vi "Progress Bar Example with User Cancel.vi"() -> ()   [LabVIEW 2015]
doc: "This example VI illustrates how to implement the process to handle situation when user cancels the operations."
uses:
  Library/New Job Status.vi
  Library/New Item Status.vi
  Library/Class/Finish.vi
  Library/Simple Progress Bar.lvlib
  Library/Class/Bar.lvclass
panel:
  out "Process Error":errorcluster
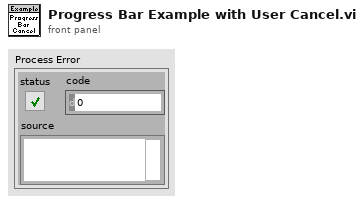
[diagram p1: front panel]
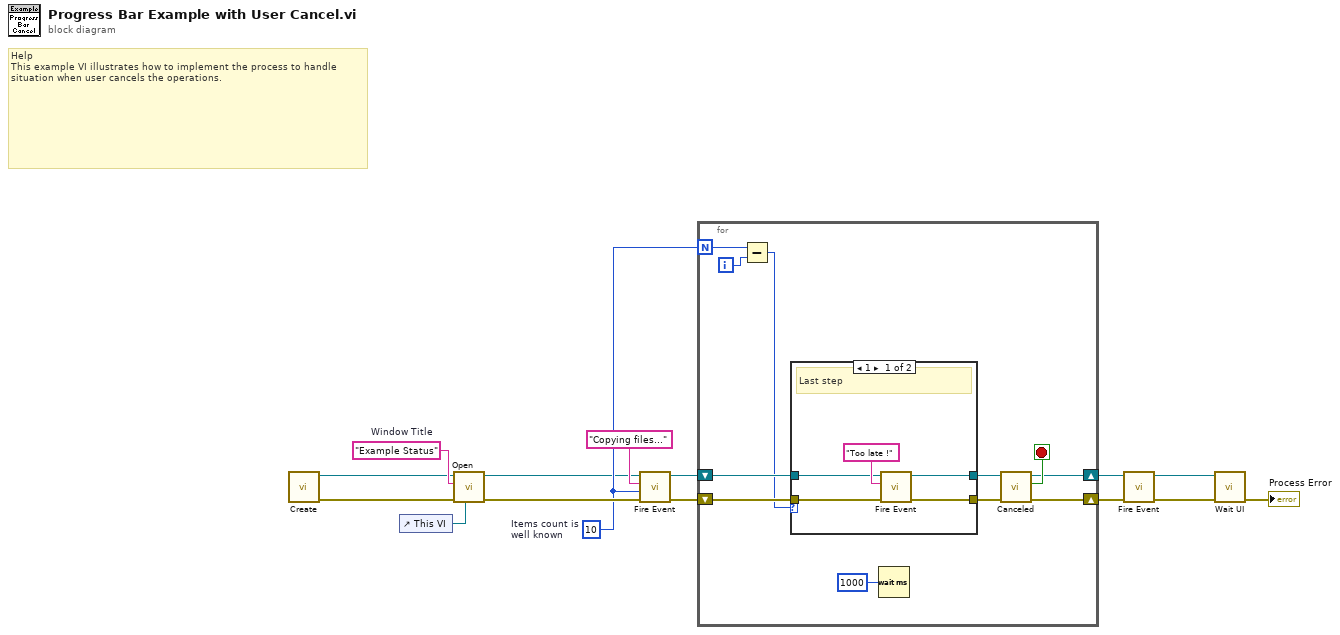
[diagram p0: block diagram]
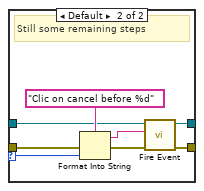
[diagram p2: hidden frame]
diagram:
  w10 = 10  # Items count is  well known
  w14 = "Example Status"  # Window Title
  # "Help\nThis example VI illustrates how to implement the process to handle situation when user cancels the operations."
  n1 = call "Create.vi"() -> ("error out"=w15:errorcluster, "Bar out"=w3:refnum<class "Bar.lvclass">)  [unwired: 10 in]
  n2 = control-ref of="This VI"() -> (w4:refnum<vi>)
  n3 = call "Open.vi"("Caller VI"=w4, "error in (no error)"=w15, "Window Title"=w14, "Bar in"=w3) -> ("error out"=w13:errorcluster, "Bar out"=w2:refnum<class "Bar.lvclass">)  [unwired: 6 in]
  n4 = call-poly "Fire Event.vi"("error in (no error)"=w13, "Items Count (unknown)"=w10, "Status"="Copying files...", "Bar in"=w2) -> ("error out"=w11:errorcluster, "Bar out"=w12:refnum<class "Bar.lvclass">)  [unwired: 6 in]
  n5 = for {
    N: w10 -> [w18]
    shift-right: [w20] -> w5
    shift-left: w11 -> [w26]
    shift-right: [w16] -> w6
    shift-left: w12 -> [w23]
    i -> [w25]
    stop <- w19 stop-if-true
    n6 = Subtract(x=w18, y=w25) -> (x-y=w22:i32)
    n7 = case shown="1" w22 {
      selector: w22 -> [_ w34]
      tunnel: w26 -> [w29 w39]
      tunnel: w23 -> [w30 w36]
      tunnel: [w28 w33] -> w21
      tunnel: [w27 w32] -> w17
      frame 1 {
        # "Last step"
        n8 = call-poly "Fire Event.vi"("error in (no error)"=w29, "Status"="Too late !" ("format string"), "Bar in"=w30) -> ("error out"=w28:errorcluster, "Bar out"=w27:refnum<class "Bar.lvclass">)  [unwired: 7 in]
      }
      frame Default {
        # "Still some remaining steps"
        n9 = Format Into String(format string="Clic on cancel before %d", error in=w39, w34) -> (resulting string=w35:string, error out=w37:errorcluster)  [unwired: 1 in]
        n10 = call-poly "Fire Event.vi"("error in (no error)"=w37, "Status"=w35, "Bar in"=w36) -> ("error out"=w33:errorcluster, "Bar out"=w32:refnum<class "Bar.lvclass">)  [unwired: 7 in]
      }
    }
    n11 = Wait (ms)(milliseconds to wait=u32 1000) -> ()  [unwired: 1 out]
    n12 = call "Canceled.vi"("error in (no error)"=w21, "Bar in"=w17) -> ("error out"=w20:errorcluster, "Canceled by user?"=w19:bool, "Bar out"=w16:refnum<class "Bar.lvclass">)  [unwired: 7 in]
  }
  n13 = call-poly "Fire Event.vi"("error in (no error)"=w5, "Bar in"=w6) -> ("error out"=w8:errorcluster, "Bar out"=w1:refnum<class "Bar.lvclass">)  [unwired: 8 in]
  n14 = call "Wait UI.vi"("error in (no error)"=w8, "Bar in"=w1) -> ("error out"=→"Process Error":errorcluster)  [unwired: 6 in, 3 out]
